vi "Cut Waveform.vi"(9 "End Time":timestamp, 10 "Start Time":timestamp, 11 "Wafeform in":waveform(dbl)) -> (3 "waveform out":waveform(dbl))   [LabVIEW 2020, in "Data Viewer.lvlib" / "Data Viewer.lvclass"]
uses:
  Data Viewer.lvclass
  <vilib>/Waveform/WDTOps.llb/WDT Get Waveform Subset DBL.vi
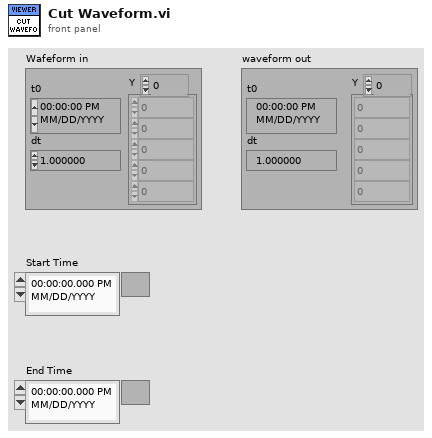
[diagram p1: front panel]
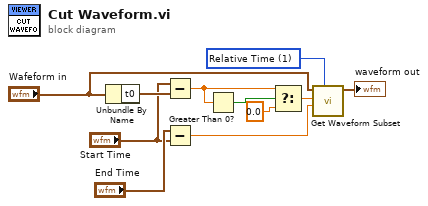
[diagram p0: block diagram]
diagram:
  w3 = u16 1 items=["Samples", "Relative Time"] ("start/duration format")
  n1 = Unbundle By Name("Wafeform in") -> ("t0"=w11:timestamp)
  n2 = Subtract(x="Start Time", y=w11) -> (x-y=w4:dbl)
  n3 = Subtract(x="End Time", y="Start Time") -> (x-y=w1:dbl)
  n4 = Greater Than 0?(x=w4) -> (x > 0?=w2:bool)
  n5 = Select(t=w4, s=w2, f=0.0) -> (s? t:f=w5:dbl)
  n6 = call-poly <vilib>:"Get Waveform Subset.vi"("start/duration format"=w3, "duration"=w1, "start samples/time"=w5, "waveform in"="Wafeform in") -> ("waveform out"=→"waveform out":waveform(dbl))  [unwired: 2 in, 3 out]
